vi "CSM Tool Name from VI.vi"(11 "VI Path":path) -> (3 "ToolName":string)   [LabVIEW 2017, in "CSM DebugTool Dialog.lvlib"]
uses:
  CSM DebugTool Dialog.lvlib
  _Shared/CSM Shared.lvlib
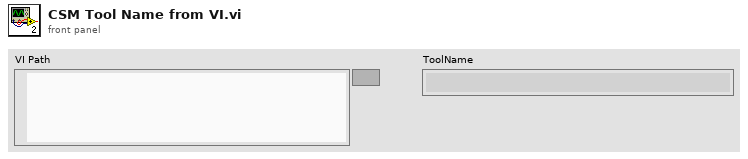
[diagram p1: front panel]
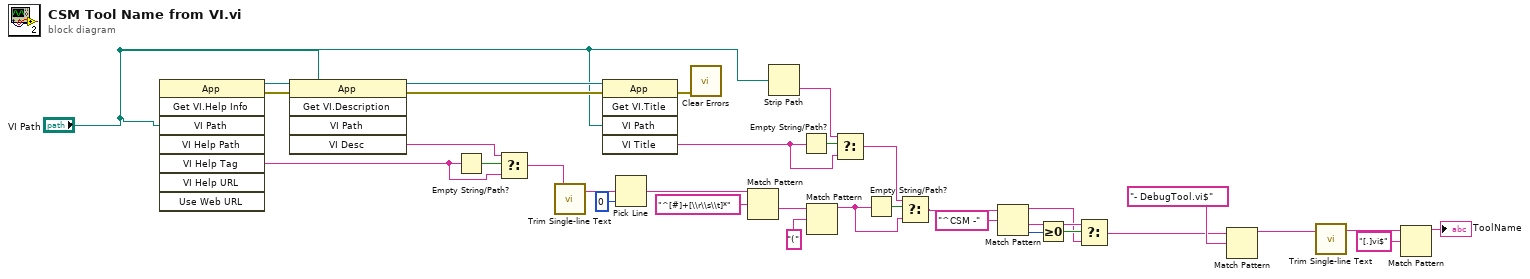
[diagram p0: block diagram]
diagram:
  n1 = invoke class="App" method="Get VI.Help Info"("VI Path"="VI Path") -> (reference out=w11:refnum<vi>, error out=w10:errorcluster, "VI Help Tag"=w8:string)  [unwired: 7 in, 5 out]
  n2 = invoke class="App" method="Get VI.Description"(reference=w11, error in=w10, "VI Path"="VI Path") -> (reference out=w33:refnum<vi>, error out=w34:errorcluster, "VI Desc"=w7:string)  [unwired: 2 in, 2 out]
  n3 = Empty String/Path?(string/path=w8) -> (empty?=w9:bool)
  n4 = Select(t=w7, s=w9, f=w8) -> (s? t:f=w6:string)
  n5 = call "Trim Single-line Text.vi"("single-line text"=w6) -> ("trimed text"=w32:string)  [unwired: 2 in]
  n6 = invoke class="App" method="Get VI.Title"(reference=w33, error in=w34, "VI Path"="VI Path") -> (error out=w14:errorcluster, "VI Title"=w4:string)  [unwired: 2 in, 3 out]
  n7 = Pick Line(multi-line string=w32, line index=0) -> (output string=w30:string)  [unwired: 1 in]
  n8 = call <vilib>:"Clear Errors.vi"("error in (no error)"=w14) -> ()  [unwired: 5 in, 2 out]
  n9 = Match Pattern(string=w30, regular expression="^[#]+[\\r\\s\\t]*") -> (after substring=w28:string)  [unwired: 1 in, 3 out]
  n10 = Strip Path(path="VI Path") -> (name=w3:string)  [unwired: 1 out]
  n11 = Empty String/Path?(string/path=w4) -> (empty?=w5:bool)
  n12 = Match Pattern(string=w28, regular expression="(") -> (before substring=w24:string)  [unwired: 1 in, 3 out]
  n13 = Select(t=w3, s=w5, f=w4) -> (s? t:f=w1:string)
  n14 = Empty String/Path?(string/path=w24) -> (empty?=w26:bool)
  n15 = Select(t=w1, s=w26, f=w24) -> (s? t:f=w17:string)
  n16 = Match Pattern(string=w17, regular expression="^CSM -") -> (before substring=w18:string, after substring=w19:string, offset past match=w21:i32)  [unwired: 1 in, 1 out]
  n17 = Greater Or Equal To 0?(x=w21) -> (x >= 0?=w20:bool)
  n18 = Select(t=w19, s=w20, f=w18) -> (s? t:f=w13:string)
  n19 = Match Pattern(string=w13, regular expression="- DebugTool.vi$") -> (before substring=w12:string)  [unwired: 1 in, 3 out]
  n20 = call "Trim Single-line Text.vi"("single-line text"=w12) -> ("trimed text"=w16:string)  [unwired: 2 in]
  n21 = Match Pattern(string=w16, regular expression="[.]vi$") -> (before substring=→"ToolName":string)  [unwired: 1 in, 3 out]
